vi "Func - FuncVI search paths.vi"(5 "cmd":enum16{"get", "set"}(ring), 6 "error in":errorcluster, 8 "user paths":path[](array[path])) -> (0 "error out":errorcluster, 2 "user paths out":path[](array[path]), 3 "search paths":path[](array[path]), 4 "base path":path)   [LabVIEW 2021]
doc: "This VI is used to define FuncVI search paths. When CalcExpress needs to call a FuncVI function, it looks through the paths specified in this VI to find the FuncVI for the called function. The full set of search paths includes predefined paths hard-coded in this VI and user-defined paths you can specify, with user-defined paths taking priority. Note that relative paths must be specified relative to the full path of this VI (including the LLB). Refer to the VI help for more details.\n\n::: CalcExpress Toolkit :::\nCopyright (c) 2000-2026 Konstantin Shifershteyn. All rights reserved."
panel:
  in  "predefined paths":path[](array[path])=[path "../FuncVI/f_math.LLB", path "../FuncVI/f_stats.LLB", path "../FuncVI/f_analys.LLB", path "../FuncVI/f_string.LLB", path "../FuncVI/f_system.LLB", path "../FuncVI/f_misc.LLB", path "../FuncVI/f_exec.LLB"]
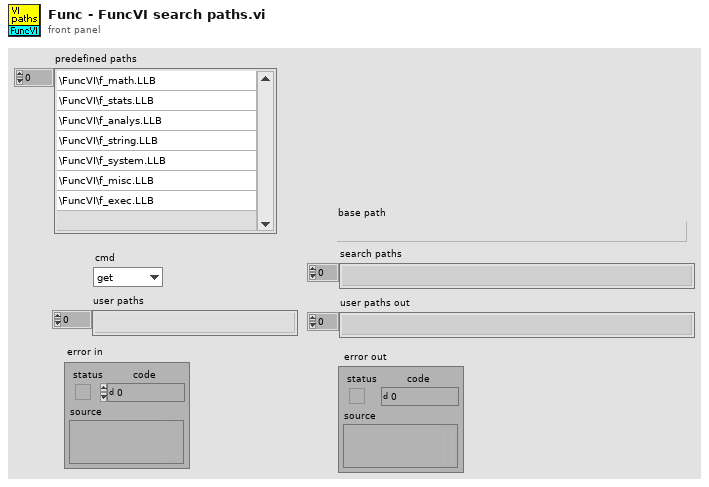
[diagram p1: front panel]
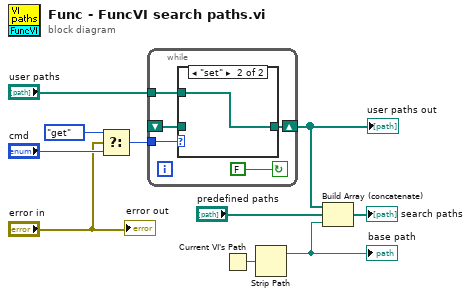
[diagram p0: block diagram]
diagram:
  n1 = Select(t=enum16{"get", "set"}."get", s="error in", f="cmd") -> (s? t:f=w4:enum16{"get", "set"})
  n2 = while {
    tunnel: w4 -> [w15]
    shift-left: _ -> [w13]
    shift-right: [w14] -> w7
    tunnel: "user paths" -> [w11]
    stop <- FALSE continue-if-true
    n3 = case shown="\"set\"" w15 {
      tunnel: [w16 w17] -> w14
      tunnel: w13 -> [w16 _]
      tunnel: w11 -> [_ w17]
      frame "get" {
      }
      frame "set" {
      }
    }
  }
  "user paths out" <- w7
  n4 = Current VI's Path() -> (path=w10:path)
  n5 = Strip Path(path=w10) -> (stripped path=w9:path)  [unwired: 1 out]
  "base path" <- w9
  n6 = Build Array (concatenate)(w7, "predefined paths", w9) -> (→"search paths":path[])
  "error out" <- "error in"
